vi "niGPS Write Waveform To File (Trajectory Script).vi"() -> ()   [LabVIEW 2016]
uses:
  <vilib>/RF Toolkits/GPS/Controls/gps version control.ctl
  <resource>/objmgr/niGPSAttribs.rc
panel:
  in  "Maximum Relative \nPower Level (dB)":dbl=10.0
  in  "Reference Power Level (dBm)":dbl=-50.0
  in  "Optimal Satellites \nUpdate Interval":dbl=30.0
  in  "Maximum Number of \nOptimal Satellites":i32=8
  in  "Initial GPS Time \nof Week":u32
  in  "Motion File Path":path=path "C:/Program Files/National Instruments/GPS/Motion files/racetrack.txt"
  in  "Stop":bool
  out "Current GPS Time of Week":dbl
  out "Satellites Selected":string
  out "Generating":bool
  in  "Waveform Scaling Factor":dbl=0.5
  in  "Receiver Location":enum32{"ECEF", "LLA "}(tab)=enum."LLA "
  in  "X":dbl=301963.44300627627 format="%#.6f"
  in  "Y":dbl=5636317.310155451 format="%#.6f"
  in  "Z":dbl=2979025.9687952213 format="%#.6f"
  in  "LLA":enum32{"Latitude", "Longitude", "Altitude"}(tab)
  in  "Lat.Degrees":dbl=27.0
  in  "Lat.Minutes":dbl=59.0
  in  "Lat.Seconds":dbl format="%#.2f"
  in  "Lat.Direction":i32(ring) items=["N", "S"]
  in  "Long.Degrees":dbl=86.0
  in  "Long.Minutes":dbl=56.0
  in  "Long.Seconds":dbl format="%#.2f"
  in  "Long.Direction":i32(ring) items=["E", "W"]
  in  "Altitude":dbl=8848.0
  in  "Initial Heading":dbl
  in  "Initial Speed":dbl
  in  "Receiver Location Format":i32(ring)=1 items=["ECEF", "LLA"]
  in  "Output GPS Binary File Path":path=path "C:/Program Files/National Instruments/GPS/Mt Everest.bin"
  in  "Ephemeris File Path":path=path "C:/Program Files/National Instruments/GPS/Ephemeris files/brdc3150.07n"
  in  "Almanac File Path":path=path "C:/Program Files/National Instruments/GPS/Almanac files/315.AL3"
  out "Error Out":errorcluster
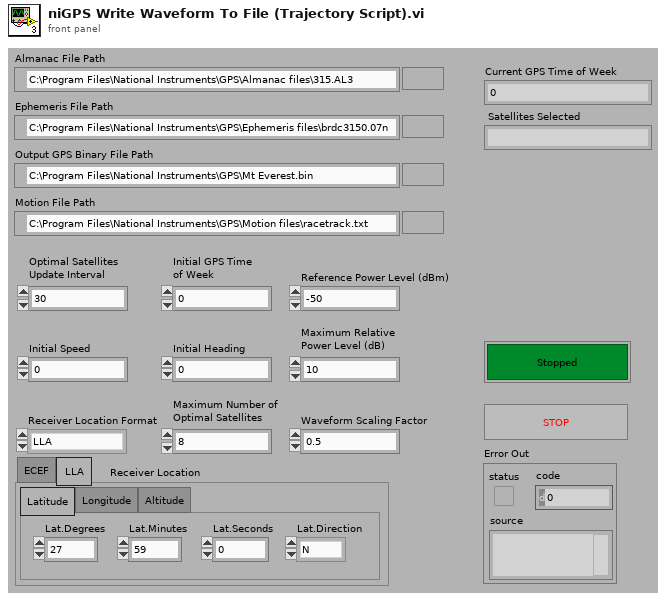
[diagram p1: front panel]
types:
  T1 = typedef "gps version control.ctl" = i32
  T2 = enum16{"open", "replace", "create", "open or create", "replace or create", "replace or create with confirmation"}
  T3 = typedef "gpsv1_refnum.ctl" = refnum<k20>
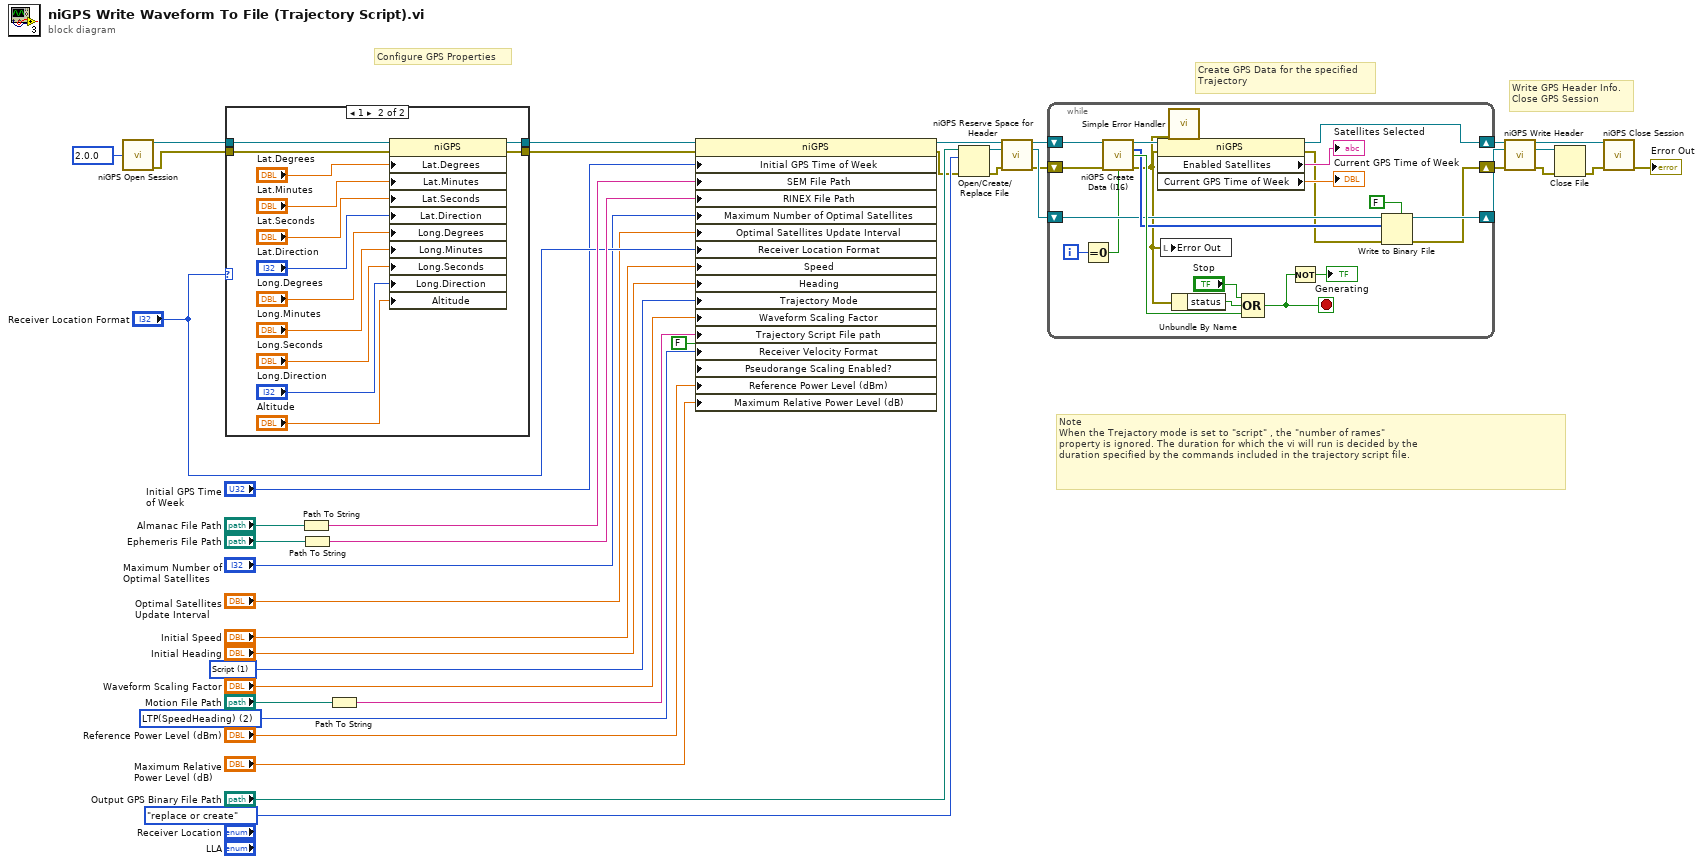
[diagram p0: block diagram]
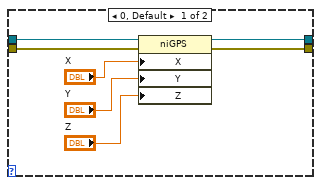
[diagram p2: hidden frame]
diagram:
  w2 = T1 20000 items=["2.0.0"=20000] ("toolkit compatibility version")
  w9 = 2 items=["ECEF", "LTP(VnVeVd)", "LTP(SpeedHeading)"] ("Receiver Velocity Format")
  w12 = 1 items=["Simple", "Script"] ("Trajectory Mode")
  # "Note\nWhen the Trejactory mode is set to \"script\" , the \"number of rames\" \nproperty is ignored. The duration for which the vi will run is decided by the \nduration specified by the commands included in the trajectory script file."
  # "Write GPS Header Info.\nClose GPS Session"
  # "Create GPS Data for the specified \nTrajectory"
  # "Configure GPS Properties"
  n1 = call <vilib>:"niGPS Open Session.vi"("toolkit compatibility version"=w2) -> ("nigps session out"=w31:T3, "error out"=w30:errorcluster)  [unwired: 2 in, 11 out]
  n2 = case shown="1" "Receiver Location Format" {
    tunnel: w31 -> [w47 w60]
    tunnel: w30 -> [w46 w59]
    tunnel: [w41 w48] -> w29
    tunnel: [w42 w49] -> w28
    frame 0, Default {
      n3 = property class="niGPS"(reference=w47, error in=w46, "X"="X", "Y"="Y", "Z"="Z") -> (reference out=w41:T3, error out=w42:errorcluster)
    }
    frame 1 {
      n4 = property class="niGPS"(reference=w60, error in=w59, "Lat.Degrees"="Lat.Degrees", "Lat.Minutes"="Lat.Minutes", "Lat.Seconds"="Lat.Seconds", "Lat.Direction"="Lat.Direction", "Long.Degrees"="Long.Degrees", "Long.Minutes"="Long.Minutes", "Long.Seconds"="Long.Seconds", "Long.Direction"="Long.Direction", "Altitude"="Altitude") -> (reference out=w48:T3, error out=w49:errorcluster)
    }
  }
  n5 = Path To String(path="Almanac File Path") -> (string=w32:string)
  n6 = Path To String(path="Ephemeris File Path") -> (string=w38:string)
  n7 = Path To String(path="Motion File Path") -> (string=w10:string)
  n8 = property class="niGPS"(reference=w29, error in=w28, "Initial GPS Time of Week"="Initial GPS Time \nof Week", "SEM File Path"=w32, "RINEX File Path"=w38, "Maximum Number of Optimal Satellites"="Maximum Number of \nOptimal Satellites", "Optimal Satellites Update Interval"="Optimal Satellites \nUpdate Interval", "Receiver Location Format"="Receiver Location Format", "Speed"="Initial Speed", "Heading"="Initial Heading", "Trajectory Mode"=w12, "Waveform Scaling Factor"="Waveform Scaling Factor", "Trajectory Script File path"=w10, "Receiver Velocity Format"=w9, "Pseudorange Scaling Enabled?"=FALSE, "Reference Power Level (dBm)"="Reference Power Level (dBm)", "Maximum Relative Power Level (dB)"="Maximum Relative \nPower Level (dB)") -> (reference out=w21:T3, error out=w25:errorcluster)
  n9 = Open/Create/Replace File(file path (use dialog)="Output GPS Binary File Path", error in=w25, operation (0:open)=T2."replace or create") -> (refnum out=w24:refnum<file>, error out=w1:errorcluster)  [unwired: 4 out]
  n10 = call <vilib>:"niGPS Reserve Space for Header.vi"("nigps session"=w21, "file refnum"=w24, "error in"=w1) -> ("nigps session out"=w20:T3, "file refnum out"=w23:refnum<file>, "error out"=w22:errorcluster)  [unwired: 10 out]
  n11 = while {
    shift-right: [w67] -> w19
    shift-left: w20 -> [w80]
    shift-right: [w70] -> w15
    shift-left: w22 -> [w79]
    shift-right: [w71] -> w17
    shift-left: w23 -> [w69]
    i -> [w66]
    stop <- w63 stop-if-true
    n12 = Equal To 0?(x=w66) -> (x = 0?=w65:bool)
    n13 = call <vilib>:"niGPS Create Data (I16).vi"("nigps session"=w80, "error in"=w79, "reset?"=w65) -> ("nigps session out"=w74:T3, "gps waveform"=w72:i16[], "done?"=w73:bool, "error out"=w61:errorcluster)  [unwired: 9 out]
    n14 = property class="niGPS"(reference=w74, error in=w61) -> (reference out=w67:T3, error out=w68:errorcluster, "Enabled Satellites"=→"Satellites Selected":string, "Current GPS Time of Week"=→"Current GPS Time of Week":dbl)
    n15 = local write "Error Out"(w61) -> ()
    n16 = call <vilib>:"Simple Error Handler.vi"("error in (no error)"=w61) -> ()  [unwired: 4 in, 5 out]
    n17 = Unbundle By Name(w61) -> ("status"=w77:bool)
    n18 = Compound Arithmetic op=OR("Stop", w77, w73) -> (w63:bool)
    n19 = Not(x=w63) -> (.not. x?=→"Generating":bool)
    n20 = Write to Binary File(file (use dialog)=w69, data=w72, error in=w68, 5:FALSE ("prepend array or string size? (T)")) -> (refnum out=w71:refnum<file>, error out=w70:errorcluster)  [unwired: 3 out]
  }
  n21 = call <vilib>:"niGPS Write Header.vi"("nigps session"=w19, "file refnum"=w17, "error in"=w15) -> ("nigps session out"=w18:T3, "file refnum out"=w16:refnum<file>, "error out"=w14:errorcluster)  [unwired: 10 out]
  n22 = Close File(refnum=w16, error in=w14) -> (error out=w39:errorcluster)  [unwired: 1 out]
  n23 = call <vilib>:"niGPS Close Session.vi"("nigps session"=w18, "error in"=w39) -> ("error out"=→"Error Out":errorcluster)  [unwired: 13 out]
